vi "PicoScopeospaSetupStreaming.vi"(0 "handle in":i16=16384, 1 "Streaming Acquisition Settings":T5={"preTriggerSamples"=0, "postTriggerSamples"=10000000, "Requested sampleInterval"=10.0, "sampleIntervalTimeUnits"=2} {"sampleIntervalTimeUnits" items=["femtoseconds", "picoseconds", "nanoseconds", "microseconds", "millseconds", "seconds"]; "postTriggerSamples" format="%_6p"; "preTriggerSamples" format="%_6p"}, 2 "Buffer and Transfer Settings":T4={"startIndex"=0, "Samples"=10000000, "Down Sample Ratio"=1, "Down-Sample Mode"=2147483648} {"Down-Sample Mode" items=["RAW none"=2147483648, "None"=0, "Aggregate"=1, "Decimate"=2, "Average"=4]; "Down Sample Ratio" step=1; "Samples" format="%_6p"}, 3 "enabled array":i16[](array[numeric])=[1, 0, 0, 0, 0, 0, 0, 0, 0, 0], 5 "Device Info":T1={"PICO_DRIVER_VERSION"="", "PICO_USB_VERSION"="", "PICO_HARDWARE_VERSION"="", "PICO_VARIANT_INFO"="", "PICO_BATCH_AND_SERIAL"="", "PICO_CAL_DATE"="", "PICO_KERNEL_VERSION"="", "PICO_DIGITAL_HARDWARE_VERSION"="", "PICO_ANALOGUE_HARDWARE_VERSION"="", "PICO_FIRMWARE_VERSION_1"="", "PICO_FIRMWARE_VERSION_2"="", "PICO_IPP_VERSION"="", "PICO_DRIVER_PATH"="", "PICO_FIRMWARE_VERSION_3"="0", "PICO_FRONT_PANEL_FIRMWARE_VERSION"="0", "Number of Channels"=0, "MSO"=TRUE}, 7 "Data Pointers In":T2={"Max Buffer Pointers"=[[[140687852109952, 80000000], [0, 55], [0, 55], [0, 55], [0, 55], [0, 55], [0, 55], [0, 55], [0, 55], [0, 55]], [[140687772090496, 80000000], [0, 55], [0, 55], [0, 55], [0, 55], [0, 55], [0, 55], [0, 55], [0, 55], [0, 55]]], "Min Buffer Pointers"=[[[0, 0], [0, 77], [0, 77], [0, 77], [0, 77], [0, 77], [0, 77], [0, 77], [0, 77], [0, 77]], [[0, 0], [0, 77], [0, 77], [0, 77], [0, 77], [0, 77], [0, 77], [0, 77], [0, 77], [0, 77]]], "StreamingDataInfo"=[[{"Channel"=0, "Down-Sample Mode"=0, "PICO_DATA_TYPE"=enum."PICO_INT16_T", "Samples"=0, "bufferIndex"=0, "startIndex"=0, "overflow"=0}], [{"Channel"=0, "Down-Sample Mode"=0, "PICO_DATA_TYPE"=enum."PICO_INT8_T", "Samples"=0, "bufferIndex"=0, "startIndex"=0, "overflow"=0}]]}, 9 "Number of Buffers":i32=3, 11 "error in (no error)":errorcluster, 12 "Auto Stop":bool) -> (4 "handle out":i16=16384, 8 "Data Pointers":T2={"Max Buffer Pointers"=[[[140687852109952, 80000000], [0, 55], [0, 55], [0, 55], [0, 55], [0, 55], [0, 55], [0, 55], [0, 55], [0, 55]], [[140687772090496, 80000000], [0, 55], [0, 55], [0, 55], [0, 55], [0, 55], [0, 55], [0, 55], [0, 55], [0, 55]], [[140687231811712, 80000000], [0, 55], [0, 55], [0, 55], [0, 55], [0, 55], [0, 55], [0, 55], [0, 55], [0, 55]]], "Min Buffer Pointers"=[[[0, 0], [0, 77], [0, 77], [0, 77], [0, 77], [0, 77], [0, 77], [0, 77], [0, 77], [0, 77]], [[0, 0], [0, 77], [0, 77], [0, 77], [0, 77], [0, 77], [0, 77], [0, 77], [0, 77], [0, 77]], [[0, 0], [0, 77], [0, 77], [0, 77], [0, 77], [0, 77], [0, 77], [0, 77], [0, 77], [0, 77]]], "StreamingDataInfo"=[[{"Channel"=0, "Down-Sample Mode"=0, "PICO_DATA_TYPE"=enum."PICO_INT16_T", "Samples"=0, "bufferIndex"=0, "startIndex"=0, "overflow"=0}], [{"Channel"=0, "Down-Sample Mode"=0, "PICO_DATA_TYPE"=enum."PICO_INT8_T", "Samples"=0, "bufferIndex"=0, "startIndex"=0, "overflow"=0}], [{"Channel"=0, "Down-Sample Mode"=0, "PICO_DATA_TYPE"=enum."PICO_INT8_T", "Samples"=0, "bufferIndex"=0, "startIndex"=0, "overflow"=0}]]}, 13 "Actual sampleInterval":T3={"sampleInterval"=10.0, "sampleIntervalTimeUnits"=2} {"sampleIntervalTimeUnits" items=["femtoseconds", "picoseconds", "nanoseconds", "microseconds", "millseconds", "seconds", ""]}, 15 "error out":errorcluster)   [LabVIEW 2010]
doc: "Setup streaming Pico data buffers and first calls to SetDataDataBuffer"
uses:
  shared/PicoBuffers.ctl
  psospa.dll
  shared/Buffer and Transfer Settings.ctl
panel:
  in  "Dummy enabled array":i16[](array[numeric])=[1, 1, 1, 1, 1, 1, 1, 1, 1, 1]
  out "Actionflag":bool=TRUE
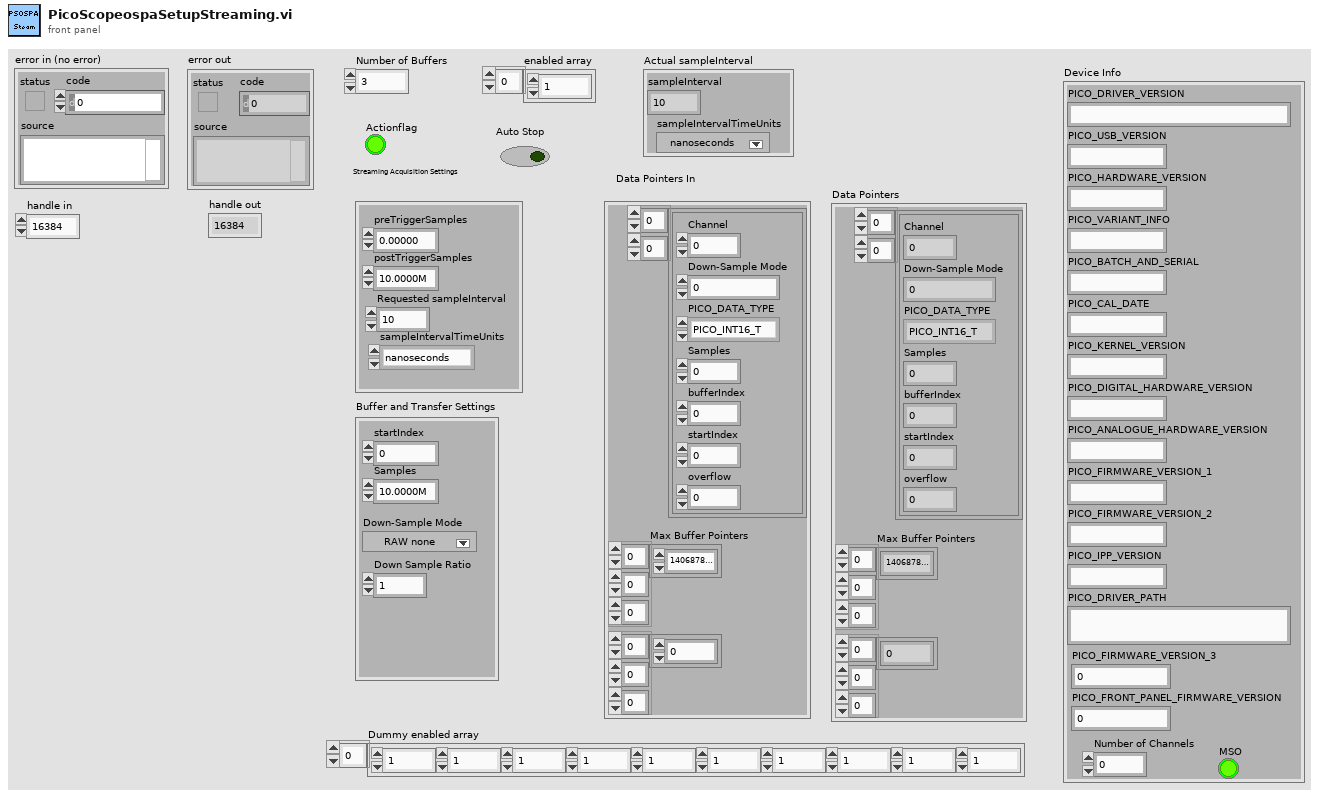
[diagram p1: front panel]
types:
  T1 = cluster{"PICO_DRIVER_VERSION":string, "PICO_USB_VERSION":string, "PICO_HARDWARE_VERSION":string, "PICO_VARIANT_INFO":string, "PICO_BATCH_AND_SERIAL":string, "PICO_CAL_DATE":string, "PICO_KERNEL_VERSION":string, "PICO_DIGITAL_HARDWARE_VERSION":string, "PICO_ANALOGUE_HARDWARE_VERSION":string, "PICO_FIRMWARE_VERSION_1":string, "PICO_FIRMWARE_VERSION_2":string, "PICO_IPP_VERSION":string, "PICO_DRIVER_PATH":string, "PICO_FIRMWARE_VERSION_3":string, "PICO_FRONT_PANEL_FIRMWARE_VERSION":string, "Number of Channels":i16, "MSO":bool}
  T2 = typedef "PicoBuffers.ctl" = cluster{"Max Buffer Pointers":u64[][][], "Min Buffer Pointers":u64[][][], "StreamingDataInfo":cluster{"Channel":u32, "Down-Sample Mode":u32, "PICO_DATA_TYPE":enum32{"PICO_INT8_T", "PICO_INT16_T", "PICO_INT32_T", "PICO_UINT32_T", "PICO_INT64_T", ""}, "Samples":i32, "bufferIndex":u64, "startIndex":i32, "overflow":i16}[][]}
  T3 = cluster{"sampleInterval":dbl, "sampleIntervalTimeUnits":u32}
  T4 = typedef "Buffer and Transfer Settings.ctl" = cluster{"startIndex":u64, "Samples":u64, "Down Sample Ratio":u64, "Down-Sample Mode":u32}
  T5 = cluster{"preTriggerSamples":u64, "postTriggerSamples":u64, "Requested sampleInterval":dbl, "sampleIntervalTimeUnits":u32}
  T6 = cluster{"Channel":u32, "Down-Sample Mode":u32, "PICO_DATA_TYPE":enum32{"PICO_INT8_T", "PICO_INT16_T", "PICO_INT32_T", "PICO_UINT32_T", "PICO_INT64_T", ""}, "Samples":i32, "bufferIndex":u64, "startIndex":i32, "overflow":i16}
  T7 = enum32{"PICO_INT8_T", "PICO_INT16_T", "PICO_INT32_T", "PICO_UINT32_T", "PICO_INT64_T", ""}
  T8 = cluster{"status":bool, "code":u32, "source":string}
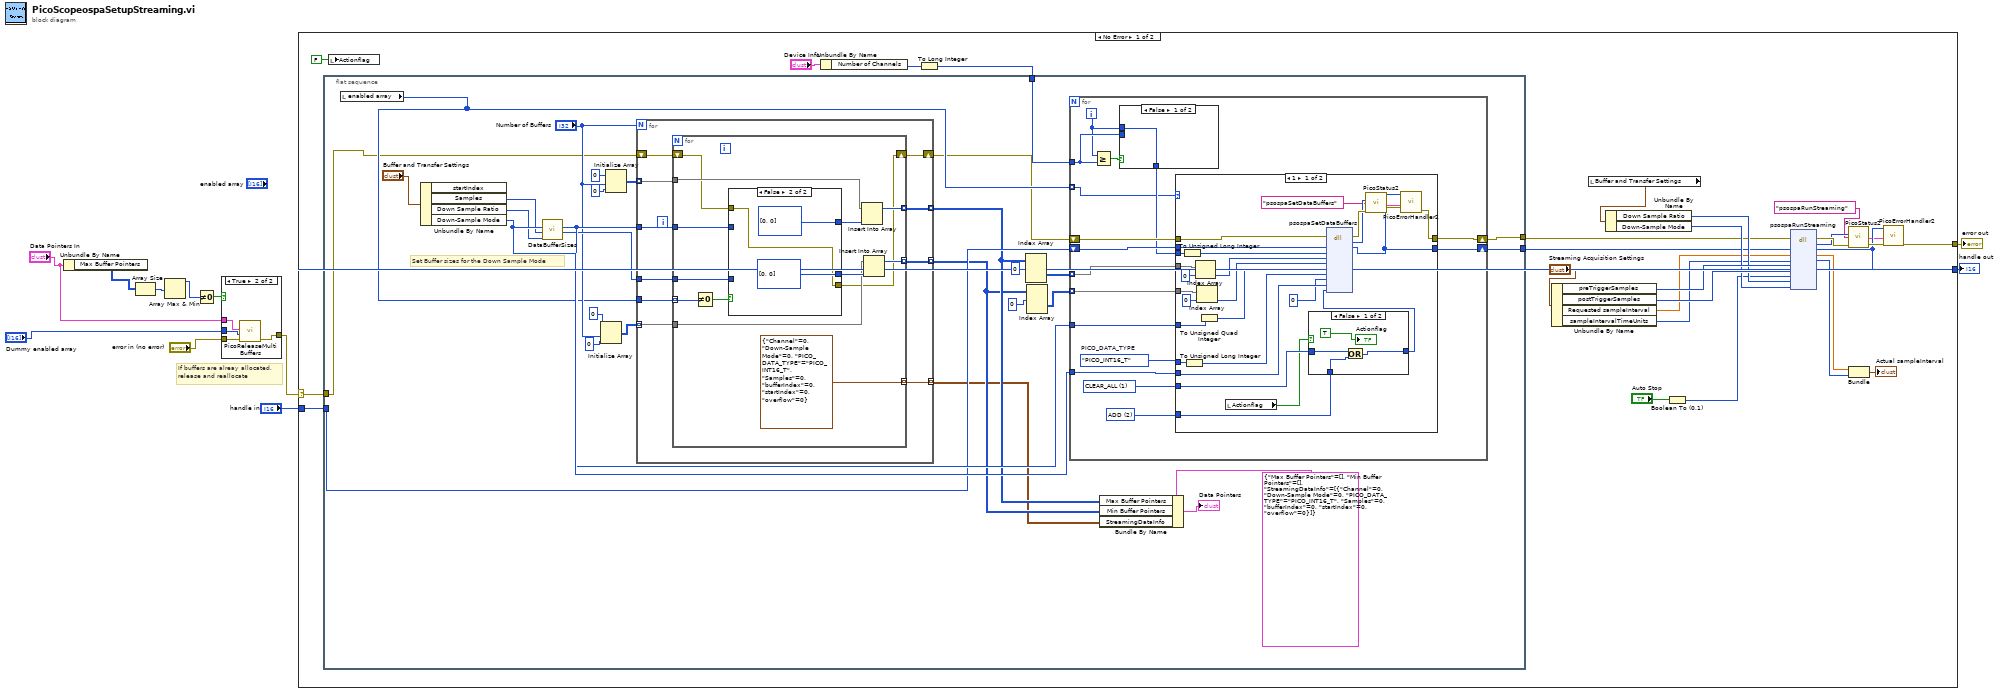
[diagram p0: block diagram]
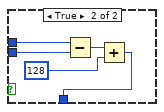
[diagram p3: hidden frame]
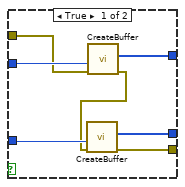
[diagram p6: hidden frame]
diagram:
  # "If buffers are alreay allocated,\nrelease and reallocate"
  n1 = Unbundle By Name("Data Pointers In") -> ("Max Buffer Pointers"=w3:u64[][][])
  n2 = Array Size(array=w3) -> (size(s)=w7:i32[])
  n3 = Array Max & Min(array=w7) -> (max value=w6:i32)  [unwired: 3 out]
  n4 = Not Equal To 0?(x=w6) -> (x != 0?=w8:bool)
  n5 = case shown="True" w8 {
    tunnel: "error in (no error)" -> [w12 w16]
    tunnel: [w12 w15] -> w4
    tunnel: "Dummy enabled array" -> [_ w14]
    tunnel: "Data Pointers In" -> [_ w13]
    frame False {
    }
    frame True {
      n6 = call "PicoReleaseMultiBuffers.vi"("error in (no error)"=w16, "Enabled array"=w14, "Data Pointers"=w13) -> ("error out"=w15:errorcluster)  [unwired: 7 in, 1 out]
    }
  }
  n7 = case shown="No Error" w4 {
    selector: w4 -> [w34 w163]
    tunnel: "handle in" -> [w33 w164]
    tunnel: [w26 w164] -> w10
    tunnel: [w27 w163] -> w9
    frame No Error {
      n8 = flat-sequence {
        tunnel: w34 -> [w46]
        tunnel: w33 -> [w57]
        tunnel: [w58] -> w32
        tunnel: [w54] -> w31
        tunnel: w19 -> [w48]
        frame #0 {
          # "Set Buffer sizes for the Down Sample Mode"
          n9 = local read "enabled array"() -> (w49:i16[])
          n10 = Unbundle By Name("Buffer and Transfer Settings") -> ("Samples"=w66:u64, "Down Sample Ratio"=w65:u64, "Down-Sample Mode"=w67:u32)  [unwired: 1 out]
          n11 = call "DataBufferSizes.vi"("Down Sample Ratio"=w65, "Number of Samples"=w66, "Down-Sample Mode"=w67) -> ("min Buffer Size"=w63:i32, "Max Buffer Size"=w64:i32)  [unwired: 7 in]
          n12 = Initialize Array(u64 0 ("element"), "Number of Buffers", 0 ("dimension size")) -> (w60:u64[][])
          n13 = Initialize Array(u64 0 ("element"), "Number of Buffers", 0 ("dimension size")) -> (w68:u64[][])
          n14 = for {
            N: "Number of Buffers" -> [_]
            tunnel: w49 -> [w138]
            tunnel: w64 -> [w139]
            tunnel: w63 -> [w137]
            tunnel: [w136] -> w53 mode=indexing
            tunnel: w68 -> [w135] mode=indexing
            tunnel: w60 -> [w134] mode=indexing
            tunnel: [w133] -> w52 mode=indexing
            tunnel: [w132] -> w47 mode=indexing
            shift-right: [w130] -> w45
            shift-left: w46 -> [w131]
            n15 = for {
              tunnel: w139 -> [w152]
              tunnel: w138 -> [w150] mode=indexing
              tunnel: w137 -> [w149]
              tunnel: [w147] -> w136 mode=indexing
              tunnel: w135 -> [w146]
              tunnel: w134 -> [w144]
              tunnel: [w143] -> w133 mode=indexing
              tunnel: [T6 {"Channel"=0, "Down-Sample Mode"=0, "PICO_DATA_TYPE"=enum."PICO_INT16_T", "Samples"=0, "bufferIndex"=0, "startIndex"=0, "overflow"=0} ("C Struture define 3")] -> w132 mode=indexing
              shift-right: [w140] -> w130
              shift-left: w131 -> [w141]
              n16 = Not Equal To 0?(x=w150) -> (x != 0?=w151:bool)
              n17 = case shown="False" w151 {
                tunnel: w152 -> [w158 _]
                tunnel: w149 -> [w159 _]
                tunnel: [w157 u64[] [0, 0]] -> w148
                tunnel: [w156 u64[] [0, 0]] -> w145
                tunnel: w141 -> [w155 w160]
                tunnel: [w153 w160] -> w140
                frame True {
                  n18 = call "CreateBuffer.vi"("error in (no error)"=w155, "Buffer size"=w158) -> ("error out"=w154:errorcluster, "Pointer and BufferSize"=w157:u64[])  [unwired: 8 in]
                  n19 = call "CreateBuffer.vi"("error in (no error)"=w154, "Buffer size"=w159) -> ("error out"=w153:errorcluster, "Pointer and BufferSize"=w156:u64[])  [unwired: 8 in]
                }
                frame False {
                }
              }
              n20 = Insert Into Array(array=w146, new element=w148) -> (w147:u64[])  [unwired: 1 in]
              n21 = Insert Into Array(array=w144, new element=w145) -> (w143:u64[])  [unwired: 1 in]
            }
          }
          n22 = Index Array(array=w53, index (dim 0)=0 ("index")) -> (element=w71:u64[][])  [unwired: 2 in]
          n23 = Index Array(array=w52, index (dim 0)=0 ("index")) -> (element=w55:u64[][])  [unwired: 2 in]
          n24 = for {
            tunnel: w67 -> [w89]
            tunnel: w64 -> [w84]
            tunnel: w49 -> [w74] mode=indexing
            tunnel: w71 -> [w83] mode=indexing
            shift-right: [w82] -> w58
            shift-left: w45 -> [w88]
            tunnel: w55 -> [w78] mode=indexing
            shift-right: [w77] -> w54
            shift-left: w57 -> [w87]
            tunnel: w48 -> [w76]
            i -> [w75]
            w79 = T7."PICO_INT16_T"  # PICO_DATA_TYPE
            w80 = u32 1 items=["NONE"=0, "CLEAR_ALL"=1, "ADD"=2, "CLEAR_THIS_DATA_BUFFER"=4096, "CLEAR_WAVEFORM_DATA_BUFFERS"=8192, "CLEAR_WAVEFORM_READ_DATA_BUFFERS"=16384] ("PicoAction 1")
            w81 = u32 2 items=["NONE"=0, "CLEAR_ALL"=1, "ADD"=2, "CLEAR_THIS_DATA_BUFFER"=4096, "CLEAR_WAVEFORM_DATA_BUFFERS"=8192, "CLEAR_WAVEFORM_READ_DATA_BUFFERS"=16384] ("PicoAction 2")
            n25 = Greater Or Equal?(x=w75, y=w76) -> (x >= y?=w86:bool)
            n26 = case shown="False" w86 {
              tunnel: [w90 w94] -> w85
              tunnel: w76 -> [_ w93]
              tunnel: w75 -> [w90 w92]
              frame False {
              }
              frame True {
                n27 = Subtract(x=w92, y=w93) -> (x-y=w91:i32)
                n28 = Add(x=w91, y=128) -> (x+y=w94:i32)
              }
            }
            n29 = case shown="1" w74 {
              tunnel: w85 -> [w111 _]
              tunnel: w88 -> [w122 w129]
              tunnel: w87 -> [w119 w128]
              tunnel: w89 -> [w116 _]
              tunnel: w79 -> [w101 _]
              tunnel: w80 -> [w106 _]
              tunnel: [w115 w129] -> w82
              tunnel: [w114 w128] -> w77
              tunnel: w84 -> [w113 _]
              tunnel: w83 -> [w107 _]
              tunnel: w81 -> [w105 _]
              tunnel: w78 -> [w97 _]
              frame 1 {
                n30 = To Unsigned Long Integer(number=w111) -> (unsigned 32bit integer=w110:u32)
                n31 = To Unsigned Long Integer(number=w101) -> (unsigned 32bit integer=w102:u32)
                n32 = Index Array(array=w107, index=0) -> (element=w108:u64)
                n33 = Index Array(array=w97, index=0) -> (element=w98:u64)
                n34 = To Unsigned Quad Integer(1:w113) -> (0:w112:u64)
                n35 = local read "Actionflag"() -> (w103:bool)
                n36 = case shown="False" w103 {
                  tunnel: w106 -> [w126 _]
                  tunnel: w105 -> [w125 w127]
                  tunnel: [w124 w127] -> w104
                  frame False {
                    n37 = Or(x=w126, y=w125) -> (x .or. y?=w124:u32)
                    "Actionflag" <- TRUE ("Actionflag")
                  }
                  frame True {
                  }
                }
                n38 = dll-call lib="psospa.dll" fn="psospaSetDataBuffers" ("ps3000.dll:_ps3000_open_unit@0")(error in=w122, "handle"=w119, "channel"=w110, "bufferMax"=w108, "bufferMin"=w98, "nSamples"=w112, "dataType"=w102, "waveform"=u64 0, "downSampleRatioMode"=w116, "action"=w104) -> (error out=w121:errorcluster, "PICO_STATUS"=w120:u32, "handle"=w114:i16)  [unwired: 10 in, 1 out]
                n39 = call "PicoStatus2.vi"("PICO source"="psospaSetDataBuffers" ("source"), "Error in"=w121, "PICO STATUS"=w120) -> ("error out"=w117:errorcluster, "PICO_STATUS out"=w96:T8)  [unwired: 5 in]
                n40 = call "PicoErrorHandler2.vi"("error in (no error)"=w117, "PICO_STATUS in"=w96, "handle In"=w114) -> ("error out"=w115:errorcluster)  [unwired: 8 in]
              }
              frame 0, Default {
              }
            }
          }
          n41 = Bundle By Name(cluster=T2 {"Max Buffer Pointers"=[], "Min Buffer Pointers"=[], "StreamingDataInfo"=[[{"Channel"=0, "Down-Sample Mode"=0, "PICO_DATA_TYPE"=enum."PICO_INT16_T", "Samples"=0, "bufferIndex"=0, "startIndex"=0, "overflow"=0}]]} ("Data Pointers"), "Max Buffer Pointers"=w53, "Min Buffer Pointers"=w52, "StreamingDataInfo"=w47) -> (→"Data Pointers":T2)
        }
      }
      n42 = local write "Actionflag"(FALSE ("Actionflag")) -> ()
      n43 = Unbundle By Name("Device Info") -> ("Number of Channels"=w18:i16)
      n44 = To Long Integer(number=w18) -> (32bit integer=w19:i32)
      n45 = Unbundle By Name("Streaming Acquisition Settings") -> ("preTriggerSamples"=w39:u64, "postTriggerSamples"=w38:u64, "Requested sampleInterval"=w30:dbl, "sampleIntervalTimeUnits"=w29:u32)
      n46 = local read "Buffer and Transfer Settings"() -> (w37:T4)
      n47 = Unbundle By Name(w37) -> ("Down Sample Ratio"=w36:u64, "Down-Sample Mode"=w35:u32)
      n48 = Boolean To (0,1)(Boolean="Auto Stop") -> (0, 1=w21:i16)
      n49 = dll-call lib="psospa.dll" fn="psospaRunStreaming" ("ps3000.dll:_ps3000_open_unit@0")(error in=w32, "handle"=w31, "sampleInterval"=w30, "sampleIntervalTimeUnits"=w29, "maxPreTriggerSamples"=w39, "maxPostPreTriggerSamples"=w38, "autoStop"=w21, "downSampleRatio"=w36, "downSampleRatioMode"=w35) -> (error out=w43:errorcluster, "PICO_STATUS"=w42:u32, "handle"=w26:i16, "sampleInterval"=w25:dbl, "sampleIntervalTimeUnits"=w24:u32)  [unwired: 7 in, 1 out]
      n50 = call "PicoStatus2.vi"("PICO source"="psospaRunStreaming" ("source"), "Error in"=w43, "PICO STATUS"=w42) -> ("error out"=w44:errorcluster, "PICO_STATUS out"=w17:T8)  [unwired: 5 in]
      n51 = Bundle("sampleInterval"=w25, "sampleIntervalTimeUnits"=w24) -> (→"Actual sampleInterval":T3)  [unwired: 1 in]
      n52 = call "PicoErrorHandler2.vi"("error in (no error)"=w44, "PICO_STATUS in"=w17, "handle In"=w26) -> ("error out"=w27:errorcluster)  [unwired: 8 in]
    }
    frame Error {
    }
  }
  "handle out" <- w10
  "error out" <- w9
